vi "Delete Top Level.vi"(8 "error in":errorcluster, 9 "Alias":string, 10 "Project Reference":refnum<vi>) -> (0 "error out":errorcluster)   [LabVIEW 2020]
doc: "Removes the TopVI tag from the project."
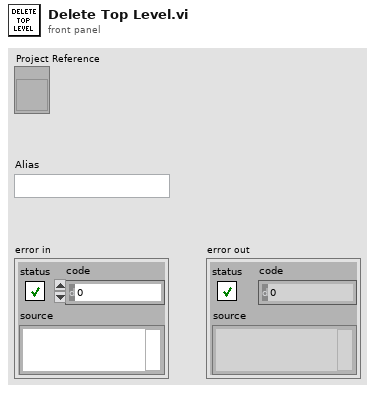
[diagram p1: front panel]
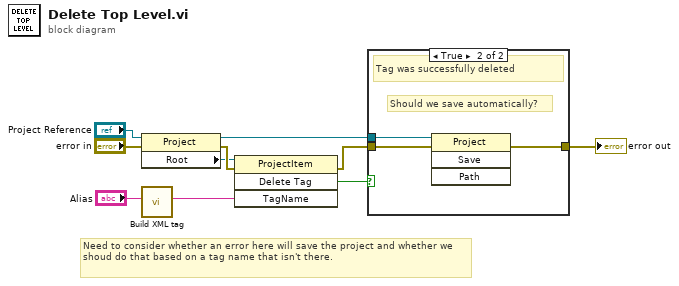
[diagram p0: block diagram]
diagram:
  # "Need to consider whether an error here will save the project and whether we shoud do that based on a tag name that isn't there."
  n1 = property class="Project"(reference="Project Reference", error in="error in") -> (reference out=w5:refnum<vi>, error out=w8:errorcluster, "Root"=w6:refnum<vi>)
  n2 = call "Build XML tag.vi"("Alias"="Alias") -> ("XML Tag"=w2:string)  [unwired: 10 in]
  n3 = invoke class="ProjectItem" method="Delete Tag"(reference=w6, error in=w8, "TagName"=w2) -> (error out=w7:errorcluster, "DeleteTag"=w1:bool)  [unwired: 1 in, 2 out]
  n4 = case shown="True" w1 {
    tunnel: [w11 w14] -> w9
    tunnel: w7 -> [w11 w13]
    tunnel: w5 -> [_ w12]
    frame False {
      # "Tag was not found/deleted"
    }
    frame True {
      # "Should we save automatically?"
      # "Tag was successfully deleted"
      n5 = invoke class="Project" method="Save"(reference=w12, error in=w13) -> (error out=w14:errorcluster)  [unwired: 2 in, 3 out]
    }
  }
  "error out" <- w9
